vi "tdms selection_T.vi"(6 "error in":errorcluster, 8 "string":string="tdms", 11 "Filename List":string[](array[string])) -> (0 "size(s)":i32, 2 "Array":string[](array[string]), 3 "Array 2":string[](array[string]), 4 "error out":errorcluster)   [LabVIEW 2018]
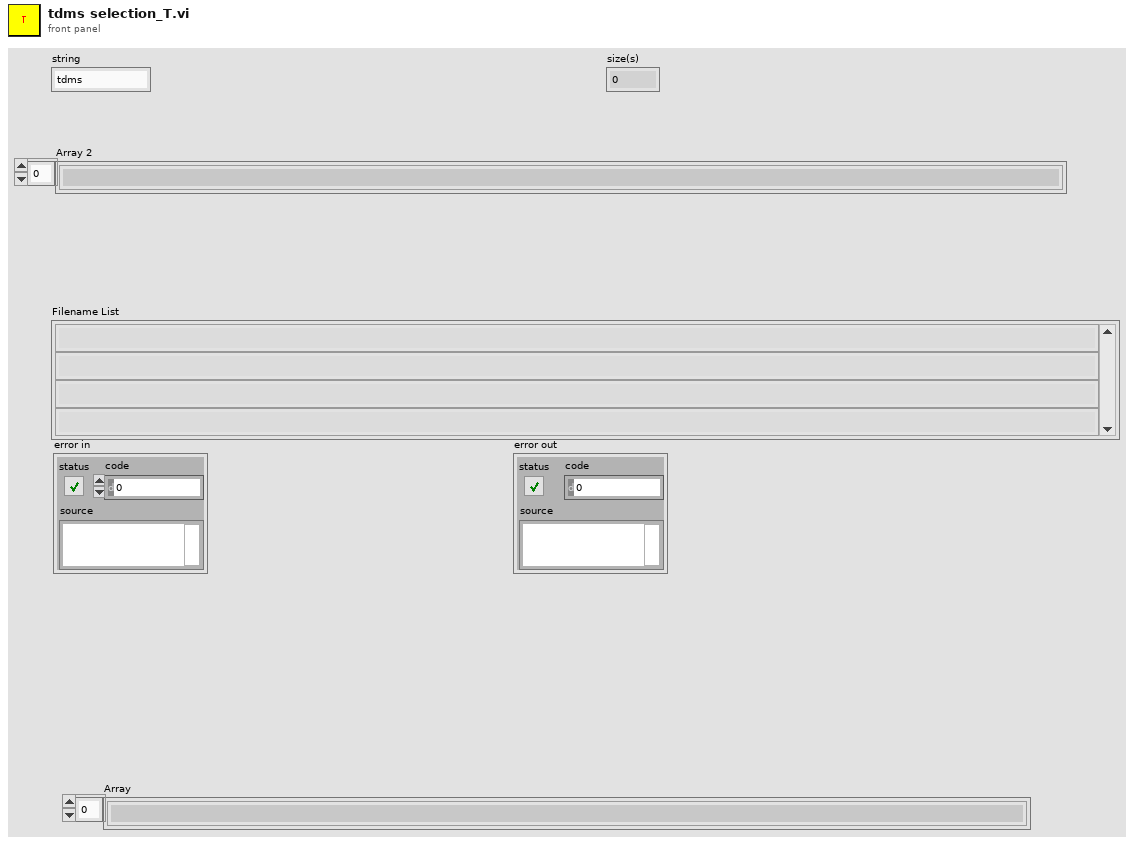
[diagram p1: front panel]
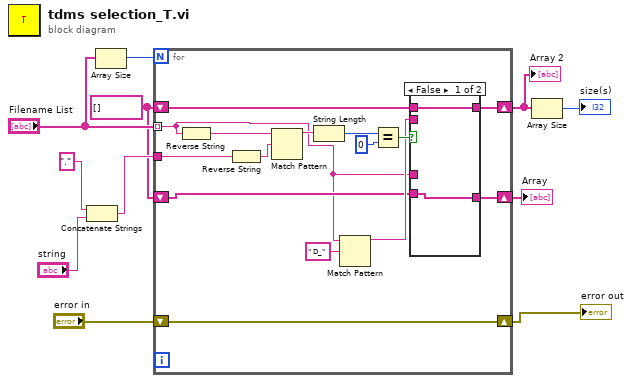
[diagram p0: block diagram]
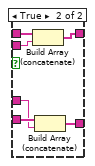
[diagram p2: hidden frame]
diagram:
  w2 = string[] []
  n1 = Concatenate Strings("." ("string"), "string") -> (w7:string)
  n2 = Array Size(array="Filename List") -> (size(s)=w11:i32)
  n3 = for {
    N: w11 -> [_]
    tunnel: "Filename List" -> [w12] mode=indexing
    shift-right: [w21] -> w9
    shift-left: w2 -> [w20]
    tunnel: w7 -> [w19]
    shift-right: [w18] -> w3
    shift-left: "error in" -> [w18]
    shift-right: [w14] -> w1
    shift-left: w2 -> [w13]
    n4 = Reverse String(1:w12) -> (0:w16:string)
    n5 = Reverse String(1:w19) -> (0:w26:string)
    n6 = Match Pattern(string=w16, regular expression=w26) -> (before substring=w25:string)  [unwired: 1 in, 3 out]
    n7 = String Length(string=w25) -> (length=w24:i32)
    n8 = Match Pattern(string=w12, regular expression=" D_") -> (before substring=w15:string)  [unwired: 1 in, 3 out]
    n9 = Equal?(x=w24, y=0) -> (x = y?=w22:bool)
    n10 = case shown="False" w22 {
      tunnel: w15 -> [_ w34]
      tunnel: [w28 w33] -> w21
      tunnel: w20 -> [w28 w32]
      tunnel: [w27 w31] -> w14
      tunnel: w13 -> [w27 w30]
      tunnel: w12 -> [_ w29]
      frame False {
      }
      frame True {
        n11 = Build Array (concatenate)(w32, w34) -> (w33:string[])
        n12 = Build Array (concatenate)(w30, w29) -> (w31:string[])
      }
    }
  }
  "Array 2" <- w9
  "error out" <- w3
  "Array" <- w1
  n13 = Array Size(array=w9) -> (size(s)=→"size(s)":i32)
